vi "T1_AOM_Manipulation.vi"(8 "Tau Step Size":dbl=2.5e-07, 9 "Numeric 2":i32, 10 "Numeric":i32, 11 "Dont Invert?":bool) -> (3 "x+y":dbl)   [LabVIEW 2024]
uses:
  <vilib>/Utility/error.llb/DialogTypeEnum.ctl
  SpinCore_API_file_location.vi
panel:
  out "output array 2":T1(array[cluster])
  out "output array":T1(array[cluster])
  in  "Instructions":T1(array[cluster])=[{"Instruct Data"=0, "Op Code"=0, "Flags"=[FALSE, FALSE, FALSE, FALSE, FALSE, FALSE, FALSE, TRUE, FALSE, FALSE, FALSE, FALSE, FALSE, FALSE, FALSE, FALSE, FALSE, FALSE, FALSE, FALSE, FALSE, FALSE, FALSE, FALSE], "Comments"="0 buffer", "Time (s)"=1e-07}, {"Instruct Data"=0, "Op Code"=0, "Flags"=[FALSE, FALSE, FALSE, FALSE, FALSE, FALSE, FALSE, TRUE, FALSE, FALSE, FALSE, FALSE, FALSE, FALSE, FALSE, FALSE, FALSE, FALSE, FALSE, FALSE, FALSE, FALSE, FALSE, FALSE], "Comments"="1 tau", "Time (s)"=1e-08}, {"Instruct Data"=0, "Op Code"=0, "Flags"=[FALSE, FALSE, TRUE, FALSE, FALSE, FALSE, FALSE, TRUE, FALSE, FALSE, FALSE, FALSE, FALSE, FALSE, FALSE, FALSE, FALSE, FALSE, FALSE, FALSE, FALSE, FALSE, FALSE, TRUE], "Comments"="2  trigger", "Time (s)"=1e-07}, {"Instruct Data"=0, "Op Code"=0, "Flags"=[FALSE, TRUE, FALSE, FALSE, FALSE, FALSE, FALSE, TRUE, FALSE, FALSE, FALSE, FALSE, FALSE, FALSE, FALSE, FALSE, FALSE, FALSE, FALSE, FALSE, FALSE, FALSE, FALSE, FALSE], "Comments"="3 aom buffer", "Time (s)"=5e-07}, {"Instruct Data"=0, "Op Code"=0, "Flags"=[FALSE, TRUE, FALSE, FALSE, FALSE, FALSE, FALSE, FALSE, FALSE, FALSE, FALSE, FALSE, FALSE, FALSE, FALSE, FALSE, FALSE, FALSE, FALSE, FALSE, FALSE, FALSE, FALSE, FALSE], "Comments"="4 inhibit off", "Time (s)"=5e-07}, {"Instruct Data"=0, "Op Code"=0, "Flags"=[FALSE, TRUE, FALSE, FALSE, FALSE, FALSE, FALSE, TRUE, FALSE, FALSE, FALSE, FALSE, FALSE, FALSE, FALSE, FALSE, FALSE, FALSE, FALSE, FALSE, FALSE, FALSE, FALSE, FALSE], "Comments"="5 AOM", "Time (s)"=5e-06}, {"Instruct Data"=0, "Op Code"=0, "Flags"=[FALSE, FALSE, FALSE, FALSE, FALSE, FALSE, FALSE, TRUE, FALSE, FALSE, FALSE, FALSE, FALSE, FALSE, FALSE, FALSE, FALSE, FALSE, FALSE, FALSE, FALSE, FALSE, FALSE, FALSE], "Comments"="6 DArk", "Time (s)"=5e-06}, {"Instruct Data"=0, "Op Code"=0, "Flags"=[TRUE, FALSE, FALSE, TRUE, FALSE, FALSE, FALSE, TRUE, FALSE, FALSE, FALSE, FALSE, FALSE, FALSE, FALSE, FALSE, FALSE, FALSE, FALSE, FALSE, FALSE, FALSE, FALSE, FALSE], "Comments"="7  pi", "Time (s)"=6.7e-08}, {"Instruct Data"=0, "Op Code"=0, "Flags"=[FALSE, TRUE, FALSE, FALSE, FALSE, FALSE, FALSE, TRUE, FALSE, FALSE, FALSE, FALSE, FALSE, FALSE, FALSE, FALSE, FALSE, FALSE, FALSE, FALSE, FALSE, FALSE, FALSE, FALSE], "Comments"="8 inhibit buffer", "Time (s)"=5e-07}, {"Instruct Data"=0, "Op Code"=0, "Flags"=[FALSE, TRUE, FALSE, FALSE, FALSE, FALSE, FALSE, FALSE, FALSE, FALSE, FALSE, FALSE, FALSE, FALSE, FALSE, FALSE, FALSE, FALSE, FALSE, FALSE, FALSE, FALSE, FALSE, FALSE], "Comments"="9 inhibit off", "Time (s)"=5e-07}, {"Instruct Data"=0, "Op Code"=6, "Flags"=[FALSE, TRUE, FALSE, FALSE, FALSE, FALSE, FALSE, TRUE, FALSE, FALSE, FALSE, FALSE, FALSE, FALSE, FALSE, FALSE, FALSE, FALSE, FALSE, FALSE, FALSE, FALSE, FALSE, FALSE], "Comments"="10 AOM", "Time (s)"=5e-06}, {"Instruct Data"=0, "Op Code"=0, "Flags"=[FALSE, TRUE, FALSE, FALSE, FALSE, FALSE, FALSE, FALSE, FALSE, FALSE, FALSE, FALSE, FALSE, FALSE, FALSE, FALSE, FALSE, FALSE, FALSE, FALSE, FALSE, FALSE, FALSE, FALSE], "Comments"="11", "Time (s)"=2.9e-06}, {"Instruct Data"=0, "Op Code"=6, "Flags"=[FALSE, FALSE, FALSE, FALSE, FALSE, FALSE, FALSE, FALSE, FALSE, FALSE, FALSE, FALSE, FALSE, FALSE, FALSE, FALSE, FALSE, FALSE, FALSE, FALSE, FALSE, FALSE, FALSE, FALSE], "Comments"="12", "Time (s)"=1e-06}] {"Time (s)" format="%.3p"; "Op Code" items=["Continue", "Stop", "Loop", "End Loop", "JSR", "RTS", "Branch", "Long Delay", "Wait"]}
  in  "# of Instructions":u32=11
  in  "clock_freq (MHz)":dbl=500.0
  # "1) MW\n2)AOM\n3)SR400 TRig\n4)I\n5)Q\n8) Inhibit\n24) Scope Trig"
  # "1"
  # "2"
  # "3"
  # "4"
  # "5"
  # "6"
  # "7"
  # "8"
  # "9"
  # "10"
  # "11"
  # "12"
  # "13"
  # "14"
  # "15"
  # "16"
  # "17"
  # "18"
  # "19"
  # "20"
  # "21"
  # "22"
  # "23"
  # "24"
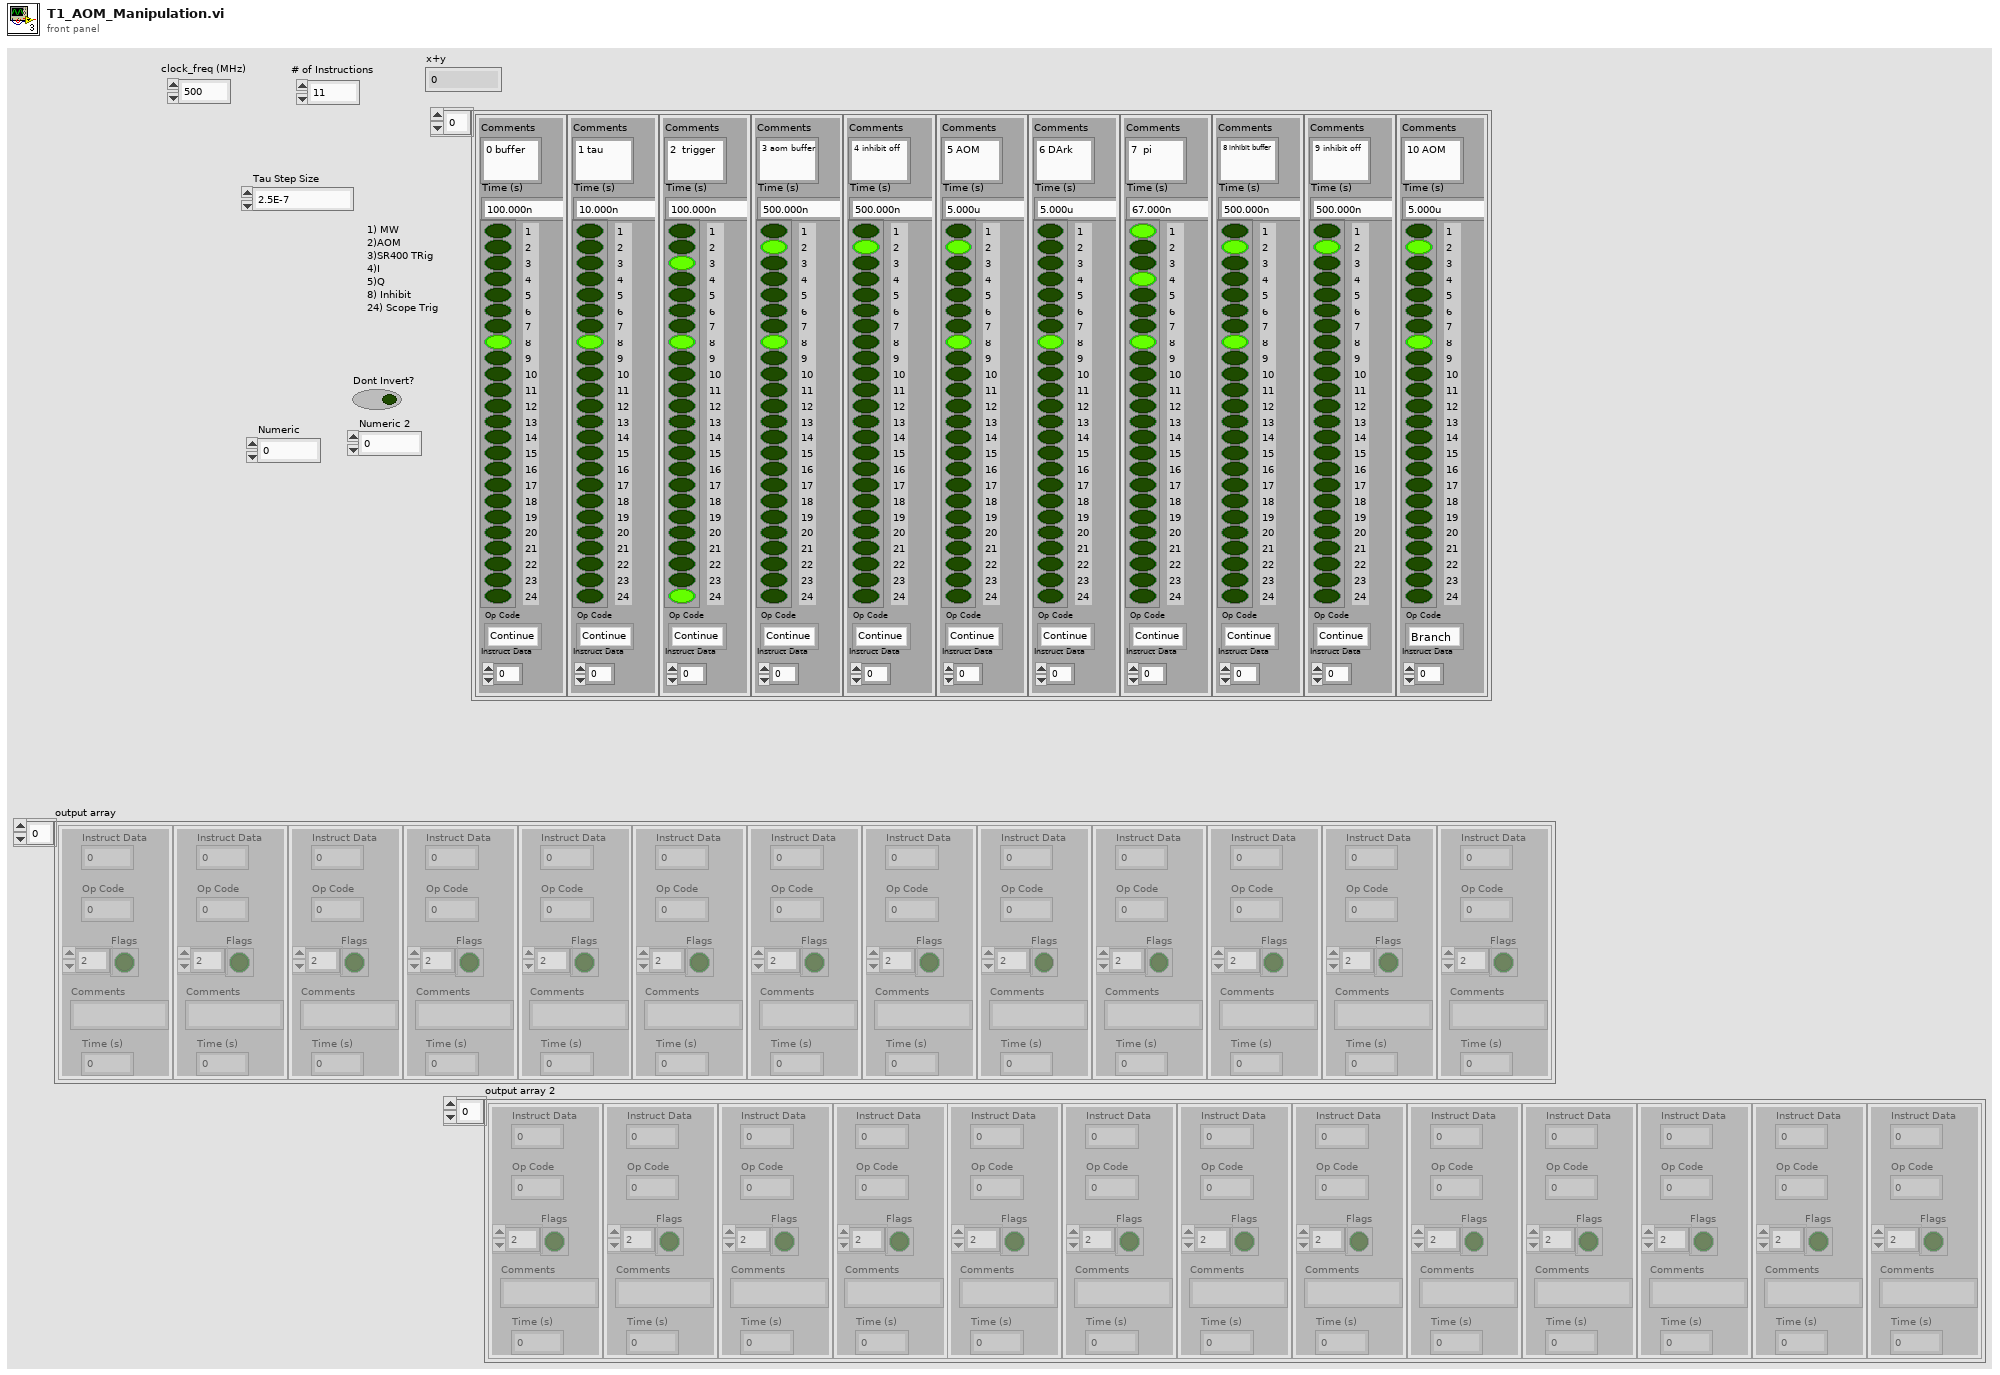
[diagram p1: front panel]
types:
  T1 = cluster{"Instruct Data":i32, "Op Code":i32, "Flags":bool[], "Comments":string, "Time (s)":dbl}[]
  T2 = typedef "DialogTypeEnum.ctl" = enum16{"no dialog", "OK message", "continue or stop message", "auto error handling dialog", "OK message + warnings", "continue/stop + warnings"}
  T3 = enum16{"Pulse Program", "Frequency Registers", "TX Phase Registers", "RX Phase Registers"}
  T4 = cluster{"Instruct Data":i32, "Op Code":i32, "Flags":bool[], "Comments":string, "Time (s)":dbl}
  T5 = cluster{"Instruct Data":i32, "Op Code":i32, "Flags":bool[], "Comments":string, dbl}
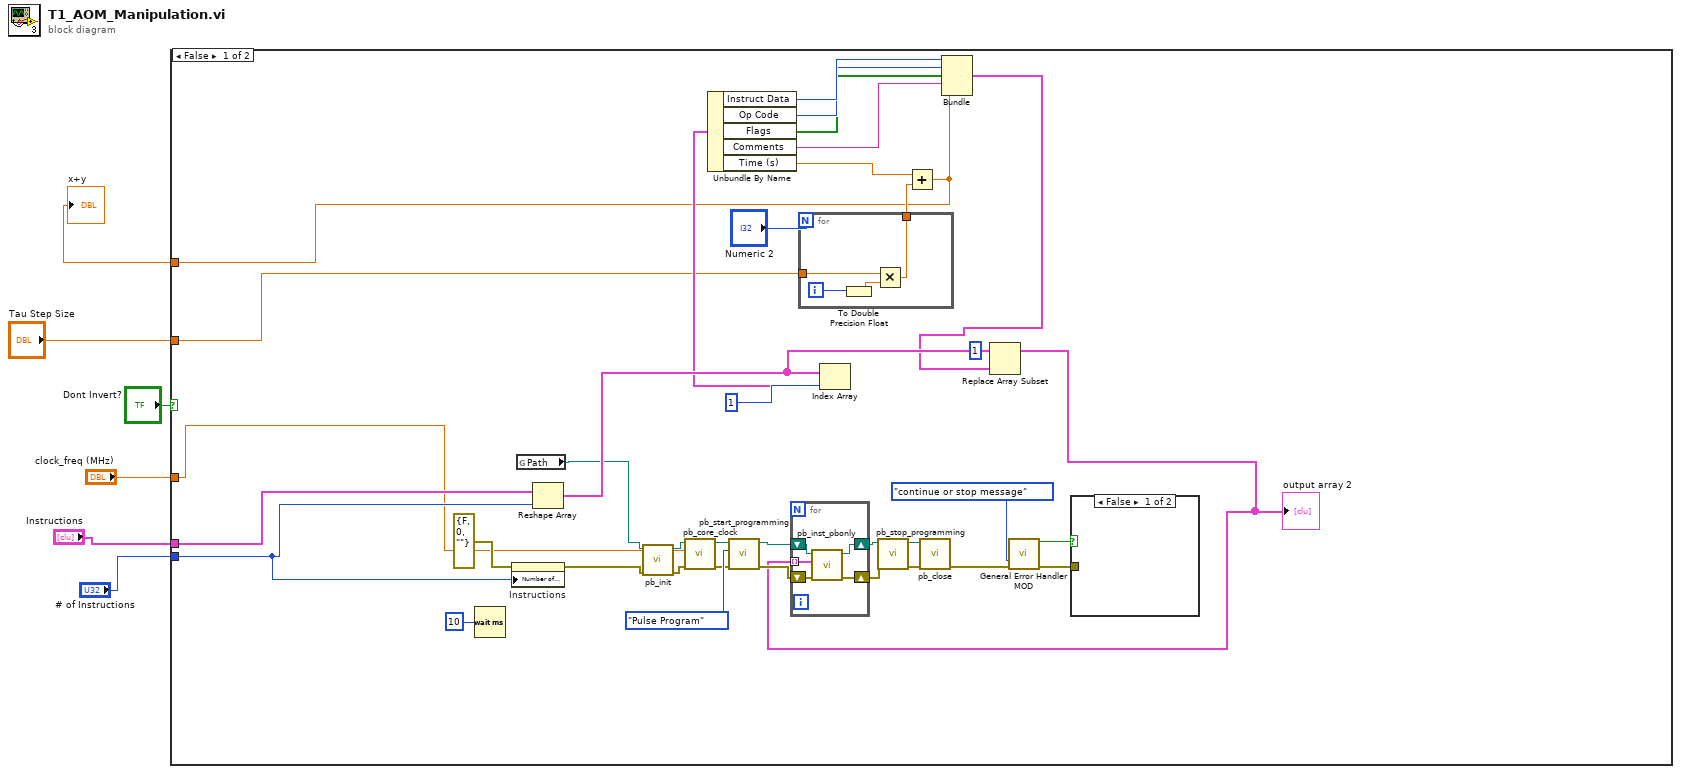
[diagram p0: block diagram]
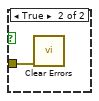
[diagram p2: hidden frame]
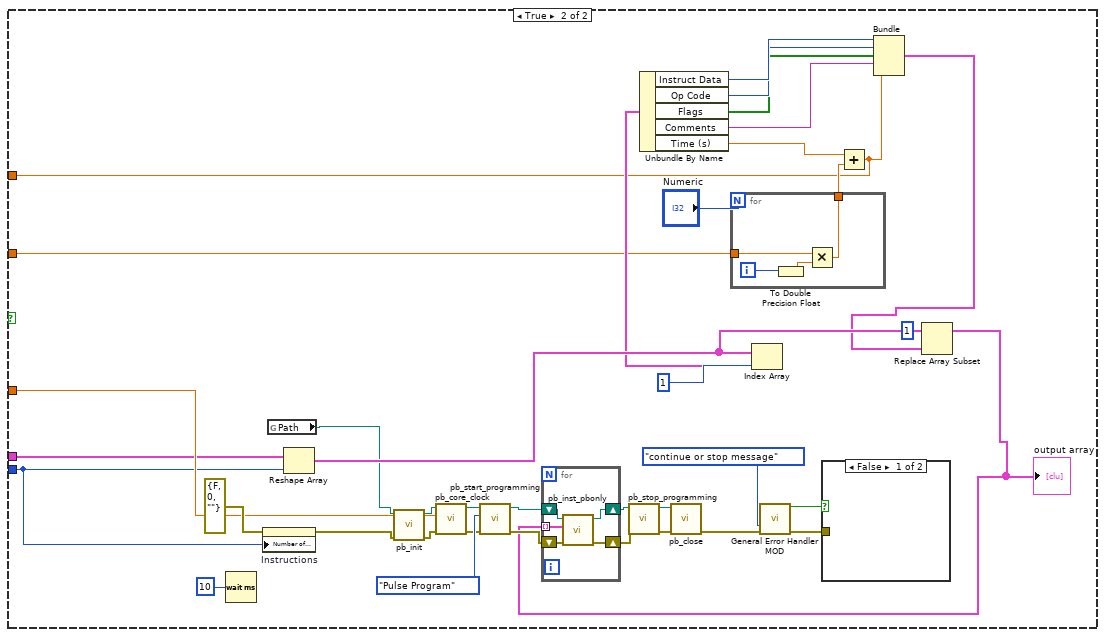
[diagram p3: hidden frame]
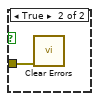
[diagram p4: hidden frame]
diagram:
  n1 = case shown="False" "Dont Invert?" {
    tunnel: "clock_freq (MHz)" -> [w8 w58]
    tunnel: "Instructions" -> [w11 w57]
    tunnel: "# of Instructions" -> [w10 w56]
    tunnel: "Tau Step Size" -> [w9 w55]
    tunnel: [w7 w54] -> w1
    frame False {
      n2 = Wait (ms)(milliseconds to wait=u32 10) -> ()  [unwired: 1 out]
      n3 = property on="Instructions" class="Arr (strict)"(error in=errorcluster {"status"=FALSE, "code"=0, "source"=""} ("error in (no error)"), "Number of Columns"=w10) -> (error out=w18:errorcluster)  [unwired: 1 in, 1 out]
      n4 = global read "SpinCore_API_file_location.vi" "Path"() -> (w19:path)
      n5 = Reshape Array "Reshape Array"(w11, w10) -> (w24:T1)
      n6 = call "pb_init.vi"("error in (no error)"=w18, "path in"=w19) -> ("error out"=w17:errorcluster, "path out"=w16:path)  [unwired: 8 in]
      n7 = call "pb_core_clock.vi"("error in (no error)"=w17, "clock_freq (MHz)"=w8, "path in"=w16) -> ("error out"=w32:errorcluster, "path out"=w33:path)  [unwired: 7 in]
      n8 = call "pb_start_programming.vi"("error in (no error)"=w32, "Device"=T3."Pulse Program", "path in"=w33) -> ("error out"=w39:errorcluster, "path out"=w43:path)  [unwired: 1 in, 6 out]
      n9 = for {
        N: "Numeric 2" -> [_]
        tunnel: [w47] -> w20
        tunnel: w9 -> [w44]
        i -> [w46]
        n10 = To Double Precision Float(number=w46) -> (double precision float=w45:dbl)
        n11 = Multiply(x=w44, y=w45) -> (x*y=w47:dbl)
      }
      n12 = Index Array "Index Array"(array=w24, index=1) -> (element=w23:T4)
      n13 = Unbundle By Name "Unbundle By Name"(w23) -> ("Instruct Data"=w29:i32, "Op Code"=w28:i32, "Flags"=w27:bool[], "Comments"=w26:string, "Time (s)"=w25:dbl)
      n14 = Add(x=w25, y=w20) -> (x+y=w7:dbl)
      n15 = Bundle("Instruct Data"=w29, "Op Code"=w28, "Flags"=w27, "Comments"=w26, w7) -> (w21:T5)  [unwired: 1 in]
      n16 = Replace Array Subset "Replace Array Subset"(array=w24, new element=w21, index=1) -> (w14:T1)
      "output array 2" <- w14
      n17 = for {
        tunnel: w14 -> [w50] mode=indexing
        shift-right: [w52] -> w41
        shift-left: w43 -> [w53]
        shift-right: [w49] -> w38
        shift-left: w39 -> [w51]
        n18 = call "pb_inst_pbonly.vi"("error in (no error)"=w51, "PB Instruction"=w50, "path in"=w53) -> ("error out"=w49:errorcluster, "path out"=w52:path)  [unwired: 2 in, 5 out]
      }
      n19 = call "pb_stop_programming.vi"("error in (no error)"=w38, "path in"=w41) -> ("error out"=w37:errorcluster, "path out"=w42:path)  [unwired: 1 in, 7 out]
      n20 = call "pb_close.vi"("error in (no error)"=w37, "path in"=w42) -> ("error out"=w31:errorcluster)  [unwired: 9 out]
      n21 = call "General Error Handler MOD.vi"("type of dialog (OK msg:1)"=DialogTypeEnum."continue or stop message", "error in (no error)"=w31) -> ("STOP?"=w34:bool, "error out"=w35:errorcluster)  [unwired: 12 out]
      n22 = case shown="False" w34 {
        tunnel: w35 -> [_ w48]
        frame False {
        }
        frame True {
          n23 = call <vilib>:"Clear Errors.vi"("error in (no error)"=w48) -> ()  [unwired: 1 in, 6 out]
        }
      }
    }
    frame True {
      n24 = Wait (ms)(milliseconds to wait=u32 10) -> ()  [unwired: 1 out]
      n25 = property on="Instructions" class="Arr (strict)"(error in=errorcluster {"status"=FALSE, "code"=0, "source"=""} ("error in (no error)"), "Number of Columns"=w56) -> (error out=w65:errorcluster)  [unwired: 1 in, 1 out]
      n26 = global read "SpinCore_API_file_location.vi" "Path"() -> (w66:path)
      n27 = Reshape Array "Reshape Array"(w57, w56) -> (w71:T1)
      n28 = call "pb_init.vi"("error in (no error)"=w65, "path in"=w66) -> ("error out"=w64:errorcluster, "path out"=w63:path)  [unwired: 8 in]
      n29 = call "pb_core_clock.vi"("error in (no error)"=w64, "clock_freq (MHz)"=w58, "path in"=w63) -> ("error out"=w79:errorcluster, "path out"=w80:path)  [unwired: 7 in]
      n30 = call "pb_start_programming.vi"("error in (no error)"=w79, "Device"=T3."Pulse Program", "path in"=w80) -> ("error out"=w86:errorcluster, "path out"=w90:path)  [unwired: 1 in, 6 out]
      n31 = for {
        N: "Numeric" -> [_]
        tunnel: [w94] -> w67
        tunnel: w55 -> [w91]
        i -> [w93]
        n32 = To Double Precision Float(number=w93) -> (double precision float=w92:dbl)
        n33 = Multiply(x=w91, y=w92) -> (x*y=w94:dbl)
      }
      n34 = Index Array "Index Array"(array=w71, index=1) -> (element=w70:T4)
      n35 = Unbundle By Name "Unbundle By Name"(w70) -> ("Instruct Data"=w76:i32, "Op Code"=w75:i32, "Flags"=w74:bool[], "Comments"=w73:string, "Time (s)"=w72:dbl)
      n36 = Add(x=w72, y=w67) -> (x+y=w54:dbl)
      n37 = Bundle("Instruct Data"=w76, "Op Code"=w75, "Flags"=w74, "Comments"=w73, w54) -> (w68:T5)  [unwired: 1 in]
      n38 = Replace Array Subset "Replace Array Subset"(array=w71, new element=w68, index=1) -> (w61:T1)
      "output array" <- w61
      n39 = for {
        tunnel: w61 -> [w97] mode=indexing
        shift-right: [w99] -> w88
        shift-left: w90 -> [w100]
        shift-right: [w96] -> w85
        shift-left: w86 -> [w98]
        n40 = call "pb_inst_pbonly.vi"("error in (no error)"=w98, "PB Instruction"=w97, "path in"=w100) -> ("error out"=w96:errorcluster, "path out"=w99:path)  [unwired: 2 in, 5 out]
      }
      n41 = call "pb_stop_programming.vi"("error in (no error)"=w85, "path in"=w88) -> ("error out"=w84:errorcluster, "path out"=w89:path)  [unwired: 1 in, 7 out]
      n42 = call "pb_close.vi"("error in (no error)"=w84, "path in"=w89) -> ("error out"=w78:errorcluster)  [unwired: 9 out]
      n43 = call "General Error Handler MOD.vi"("type of dialog (OK msg:1)"=DialogTypeEnum."continue or stop message", "error in (no error)"=w78) -> ("STOP?"=w81:bool, "error out"=w82:errorcluster)  [unwired: 12 out]
      n44 = case shown="False" w81 {
        tunnel: w82 -> [_ w95]
        frame False {
        }
        frame True {
          n45 = call <vilib>:"Clear Errors.vi"("error in (no error)"=w95) -> ()  [unwired: 1 in, 6 out]
        }
      }
    }
  }
  "x+y" <- w1
